vi "FuncVI_Sub - Probe - Set Window Position - Auto .vi"(7 "Master VI Ref":refnum<vi>, 8 "error in":errorcluster, 9 "Window Position":cluster{"x":i16, "y":i16}={"x"=32767, "y"=32767}, 11 "Probe VI Ref":refnum<vi>) -> (0 "error out":errorcluster, 3 "dup Probe VI Ref":refnum<vi>)   [LabVIEW 2021]
doc: "::: CalcExpress Toolkit :::\nCopyright (c) 2000-2026 Konstantin Shifershteyn. All rights reserved."
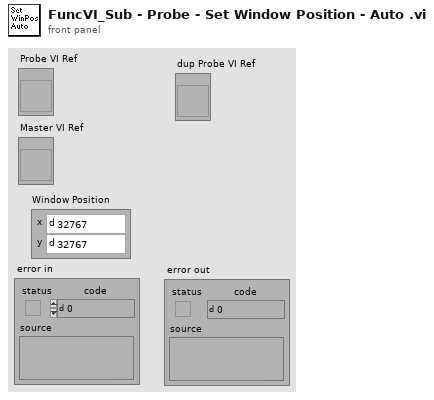
[diagram p1: front panel]
types:
  T1 = typedef "LVAllMonitorsDisplayTypeDef.ctl" = cluster{"Bounds":cluster{"Left":i16, "Top":i16, "Right":i16, "Bottom":i16}, "Depth":i16}[]
  T2 = enum32{"Invalid", "Standard", "Closed", "Hidden", "Minimized", "Maximized"}[]
  T3 = enum32{"Invalid", "Standard", "Closed", "Hidden", "Minimized", "Maximized"}
  T4 = typedef "LVRectTypeDef.ctl" = cluster{"Left":i16, "Top":i16, "Right":i16, "Bottom":i16}
  T5 = cluster{"Bounds":cluster{"Left":i16, "Top":i16, "Right":i16, "Bottom":i16}, "Depth":i16}
  T6 = cluster{"Left":i16, "Top":i16, "Right":i16, "Bottom":i16}
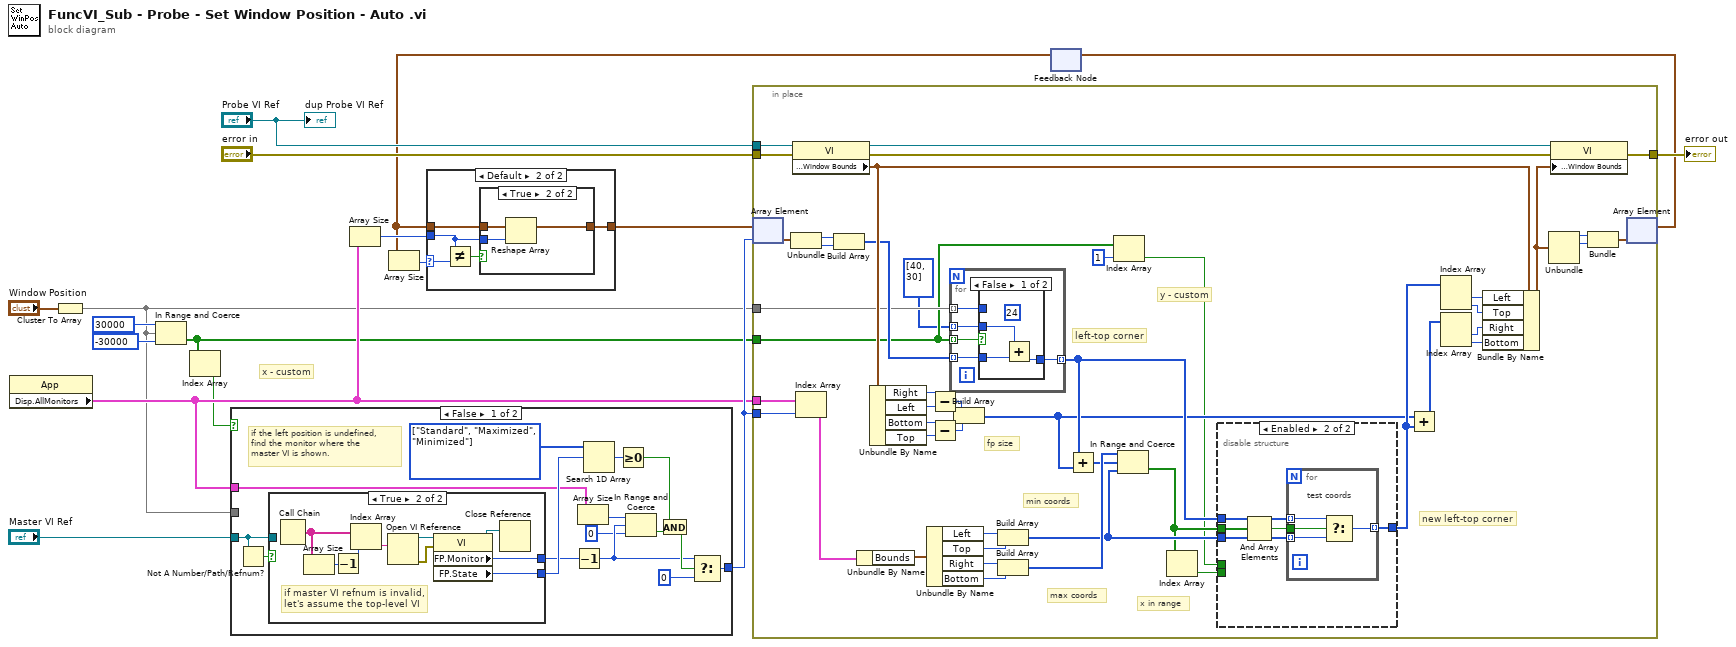
[diagram p0: block diagram]
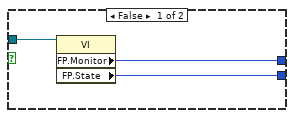
[diagram p2: hidden frame]
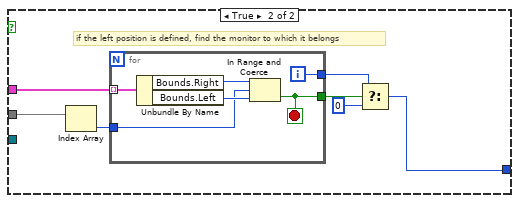
[diagram p3: hidden frame]
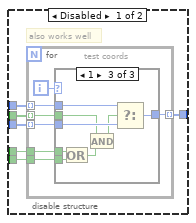
[diagram p4: hidden frame]
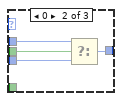
[diagram p6: hidden frame]
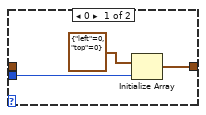
[diagram p8: hidden frame]
diagram:
  # "x - custom"
  n1 = property class="App"() -> ("Disp.AllMonitors"=w6:T1)  [unwired: 2 in, 2 out]
  n2 = Cluster To Array(cluster="Window Position") -> (array=w1:i16[])
  n3 = In Range and Coerce(upper limit=i16 30000 ("x"), x=w1, lower limit=i16 -30000 ("x")) -> (In Range?=w3:bool[])  [unwired: 1 out]
  n4 = Index Array(array=w3) -> (element=w2:bool)  [unwired: 1 in]
  n5 = case shown="False" w2 {
    tunnel: "Master VI Ref" -> [w32 _]
    tunnel: [w24 w45] -> w7
    tunnel: w6 -> [w20 w51]
    tunnel: w1 -> [_ w50]
    frame False {
      w30 = T2 [enum."Standard", enum."Maximized", enum."Minimized"] items=["Invalid", "Standard", "Closed", "Hidden", "Minimized", "Maximized"]
      # "if the left position is undefined,\nfind the monitor where the\nmaster VI is shown."
      n6 = Not A Number/Path/Refnum?(number/path/refnum=w32) -> (NaN/Path/Refnum?=w31:bool)
      n7 = case shown="True" w31 {
        tunnel: w32 -> [w35 _]
        tunnel: [w34 w37] -> w26
        tunnel: [w33 w36] -> w29
        frame False {
          n8 = property class="VI"(reference=w35) -> ("FP.Monitor"=w34:u16, "FP.State"=w33:T3)  [unwired: 1 in, 2 out]
        }
        frame True {
          # "if master VI refnum is invalid, \nlet's assume the top-level VI"
          n9 = Call Chain() -> (call chain=w44:string[])
          n10 = Array Size(array=w44) -> (size(s)=w43:i32)
          n11 = Decrement(x=w43) -> (x-1=w42:i32)
          n12 = Index Array(array=w44, index=w42) -> (element=w41:string)
          n13 = Open VI Reference(vi path=w41) -> (vi reference=w40:refnum<vi>, error out=w39:errorcluster)  [unwired: 5 in]
          n14 = property class="VI"(reference=w40, error in=w39) -> (reference out=w38:refnum<vi>, "FP.Monitor"=w37:u16, "FP.State"=w36:T3)  [unwired: 1 out]
          n15 = Close Reference(reference=w38) -> ()  [unwired: 1 in, 1 out]
        }
      }
      n16 = Decrement(x=w26) -> (x-1=w22:u16)
      n17 = Array Size(array=w20) -> (size(s)=w23:i32)
      n18 = Search 1D Array(1D array=w30, element=w29) -> (index of element=w28:i32)  [unwired: 1 in]
      n19 = Greater Or Equal To 0?(x=w28) -> (x >= 0?=w18:bool)
      n20 = In Range and Coerce(upper limit=w23, x=w22, lower limit=0) -> (In Range?=w19:bool)  [unwired: 1 out]
      n21 = And(x=w18, y=w19) -> (x .and. y?=w27:bool)
      n22 = Select(t=w22, s=w27, f=u16 0) -> (s? t:f=w24:u16)
    }
    frame True {
      # "if the left position is defined, find the monitor to which it belongs"
      n23 = Index Array(array=w50) -> (element=w49:i16)  [unwired: 1 in]
      n24 = for {
        tunnel: w51 -> [w57] mode=indexing
        tunnel: w49 -> [w54]
        tunnel: [w53] -> w48
        tunnel: [w52] -> w47
        i -> [w52]
        stop <- w53 stop-if-true
        n25 = Unbundle By Name(w57) -> ("Bounds.Right"=w55:i16, "Bounds.Left"=w56:i16)
        n26 = In Range and Coerce(upper limit=w55, x=w54, lower limit=w56) -> (In Range?=w53:bool)  [unwired: 1 out]
      }
      n27 = Select(t=w47, s=w48, f=0) -> (s? t:f=w45:i32)
    }
  }
  n28 = Array Size(array=w6) -> (size(s)=w12:i32)
  n29 = feedback #1() -> (w11:cluster{"left":i16, "top":i16}[])  [unwired: 1 in]
  n30 = Array Size(array=w11) -> (size(s)=w10:i32)
  n31 = case shown="Default" w10 {
    selector: w10 -> [_ w63]
    tunnel: w12 -> [w60 w61]
    tunnel: [w59 w64] -> w9
    tunnel: w11 -> [_ w65]
    frame 0 {
      n32 = Initialize Array(cluster{"left":i16, "top":i16} {"left"=0, "top"=0} ("Window Position"), w60) -> (w59:cluster{"left":i16, "top":i16}[])
    }
    frame Default {
      n33 = Not Equal?(x=w61, y=w63) -> (x != y?=w62:bool)
      n34 = case shown="True" w62 {
        tunnel: w65 -> [w66 w69]
        tunnel: [w66 w68] -> w64
        tunnel: w61 -> [_ w67]
        frame False {
        }
        frame True {
          n35 = Reshape Array "Reshape Array"(w69, w67) -> (w68:cluster{"left":i16, "top":i16}[])
        }
      }
    }
  }
  n36 = in-place {
    in-place-border: [w106] -> w17
    in-place-border: w1 -> [w84]
    in-place-border: "error in" -> [w105]
    in-place-border: "Probe VI Ref" -> [w104]
    in-place-border: w6 -> [w91]
    in-place-border: w7 -> [w90]
    in-place-border: w3 -> [w71]
    # "x in range"
    # "y - custom"
    # "new left-top corner"
    # "left-top corner"
    # "fp size"
    # "min coords"
    # "max coords"
    n37 = in-place-array #2(w9, w7) -> (w87:cluster{"left":i16, "top":i16})
    n38 = Unbundle(w87) -> ("left"=w86:i16, "top"=w85:i16)
    n39 = property class="VI"(reference=w104, error in=w105) -> (reference out=w109:refnum<vi>, error out=w107:errorcluster, "Front Panel Window:Window Bounds"=w108:T4)
    n40 = Index Array(array=w91, index=w90) -> (element=w89:T5)
    n41 = Build Array(w86, w85) -> (w97:i16[])
    n42 = Unbundle By Name(w89) -> ("Bounds"=w103:T6)
    n43 = Unbundle By Name(w108) -> ("Right"=w115:i16, "Left"=w114:i16, "Bottom"=w113:i16, "Top"=w112:i16)
    n44 = Unbundle By Name(w103) -> ("Left"=w102:i16, "Top"=w101:i16, "Right"=w92:i16, "Bottom"=w96:i16)
    n45 = Subtract(x=w115, y=w114) -> (x-y=w111:i16)
    n46 = Subtract(x=w113, y=w112) -> (x-y=w110:i16)
    n47 = for {
      tunnel: w84 -> [w153] mode=indexing
      tunnel: [w155] -> w81 mode=indexing
      tunnel: w97 -> [w154] mode=indexing
      tunnel: w71 -> [w152] mode=indexing
      tunnel: i16[] [40, 30] ("Window Position") -> [w151] mode=indexing
      n48 = case shown="False" w152 {
        tunnel: [w157 w159] -> w155
        tunnel: w154 -> [w158 _]
        tunnel: w153 -> [_ w159]
        tunnel: w151 -> [w156 _]
        frame False {
          (unwired) i16 24 ("y")
          n49 = Add(x=w156, y=w158) -> (x+y=w157:i16)
        }
        frame True {
        }
      }
    }
    n50 = Build Array(w111, w110) -> (w80:i16[])
    n51 = Build Array(w102, w101) -> (w82:i16[])
    n52 = Build Array(w92, w96) -> (w83:i16[])
    n53 = Add(x=w81, y=w80) -> (x+y=w79:i16[])
    n54 = Index Array(array=w71, index=1) -> (element=w72:bool)
    n55 = In Range and Coerce(upper limit=w83, x=w79, lower limit=w82) -> (In Range?=w78:bool[])  [unwired: 1 out]
    n56 = Index Array(array=w78) -> (element=w73:bool)  [unwired: 1 in]
    n57 = disable-structure shown="Enabled" {
      disable-tunnel: [w121 w146] -> w93
      disable-tunnel: w82 -> [w120 w145]
      disable-tunnel: w81 -> [w119 w144]
      disable-tunnel: w78 -> [w118 w143]
      disable-tunnel: w73 -> [w117 _]
      disable-tunnel: w72 -> [w116 _]
      frame Disabled {
        # "also works well"
        n58 = for {
          tunnel: w118 -> [w124] mode=indexing
          tunnel: w119 -> [w128] mode=indexing
          tunnel: [w126] -> w121 mode=indexing
          tunnel: w120 -> [w127] mode=indexing
          tunnel: w117 -> [w123]
          tunnel: w116 -> [w122]
          i -> [w125]
          # "test coords"
          n59 = case shown="1" w125 {
            tunnel: w128 -> [_ w133 w141]
            tunnel: w127 -> [w129 w132 w140]
            tunnel: [w129 w131 w139] -> w126
            tunnel: w124 -> [_ w130 w138]
            tunnel: w123 -> [_ _ w135]
            tunnel: w122 -> [_ _ w134]
            frame Default {
            }
            frame 0 {
              n60 = Select(t=w133, s=w130, f=w132) -> (s? t:f=w131:i16)
            }
            frame 1 {
              n61 = Or(x=w134, y=w135) -> (x .or. y?=w136:bool)
              n62 = And(x=w138, y=w136) -> (x .and. y?=w137:bool)
              n63 = Select(t=w141, s=w137, f=w140) -> (s? t:f=w139:i16)
            }
          }
        }
      }
      frame Enabled {
        n64 = And Array Elements(Boolean array=w143) -> (logical AND=w142:bool)
        n65 = for {
          tunnel: w142 -> [w147]
          tunnel: w144 -> [w150] mode=indexing
          tunnel: [w148] -> w146 mode=indexing
          tunnel: w145 -> [w149] mode=indexing
          # "test coords"
          n66 = Select(t=w150, s=w147, f=w149) -> (s? t:f=w148:i16)
        }
      }
    }
    n67 = Add(x=w80, y=w93) -> (x+y=w100:i16[])
    n68 = Index Array(array=w93) -> (element #1=w99:i16, element #2=w95:i16)  [unwired: 2 in]
    n69 = Index Array(array=w100) -> (element #1=w98:i16, element #2=w94:i16)  [unwired: 2 in]
    n70 = Bundle By Name(cluster=w108, "Left"=w99, "Top"=w95, "Right"=w98, "Bottom"=w94) -> (w77:T4)
    n71 = Unbundle(w77) -> ("Left"=w76:i16, "Top"=w75:i16)  [unwired: 2 out]
    n72 = property class="VI"(reference=w109, error in=w107, "Front Panel Window:Window Bounds"=w77) -> (error out=w106:errorcluster)  [unwired: 1 out]
    n73 = Bundle("Left"=w76, "Top"=w75) -> (w88:cluster{"Left":i16, "Top":i16})  [unwired: 1 in]
    n74 = in-place-array #2(w88) -> (w8:cluster{"left":i16, "top":i16}[])  [unwired: 1 out]
  }
  "error out" <- w17
  n75 = feedback-in #1(w8) -> ()
  "dup Probe VI Ref" <- "Probe VI Ref"
